vi "SA save Screenshot.vi"(8 "error in (no error)":errorcluster caption="에러 입력(에러 없음)", 10 "File Name":string, 11 "Instrument Manager 입력":refnum<class "Instrument Manager.lvclass">) -> (0 "error out":errorcluster caption="에러 출력", 3 "Instrument Manager 출력":refnum<class "Instrument Manager.lvclass">)   [LabVIEW 2023, in "Instrument Manager.lvclass"]
uses:
  Instrument Manager.lvclass
  Instrument Manager.lvclass/Instrument Manager.ctl
  Module/Spectrum Analyzer/Interface_Spectrum/Interface_Spectrum.lvclass
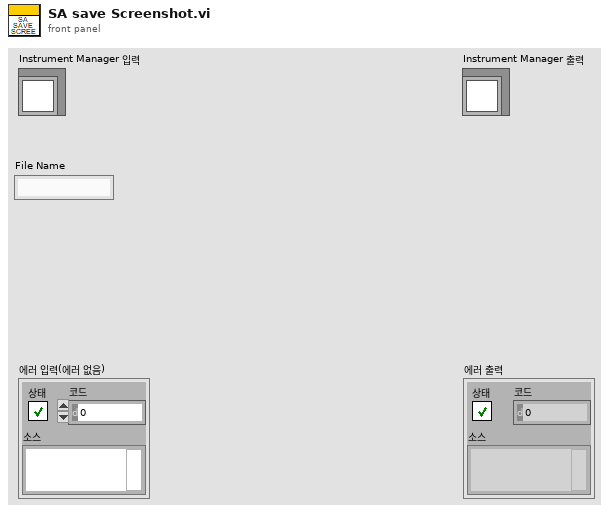
[diagram p1: front panel]
types:
  T1 = cluster{"Anritsu Call Box":refnum<class "Anritsu Call Box.lvclass">, "Spectrum Analyzer":refnum<class "Interface_Spectrum.lvclass">, "RF Switch Box":refnum<class "RF Filter Box.lvclass">, "Turn Table":refnum<class "Interface - Turn Table.lvclass">, "Mast":refnum<class "Interface - Mast.lvclass">, "3D Controller":refnum<class "Interface_3D Controller.lvclass">}
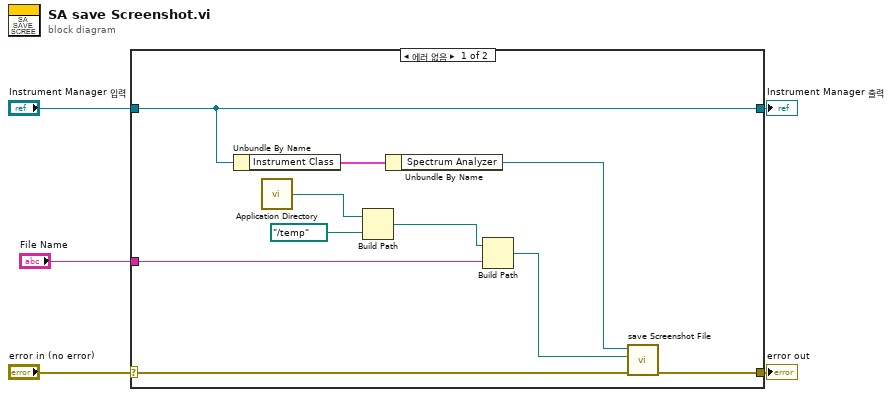
[diagram p0: block diagram]
diagram:
  n1 = case shown="에러 없음" "error in (no error)" {
    selector: "error in (no error)" -> [w12 w17]
    tunnel: [w11 w17] -> w4
    tunnel: [w10 w16] -> w2
    tunnel: "Instrument Manager 입력" -> [w10 w16]
    tunnel: "File Name" -> [w13 _]
    frame No Error {
      n2 = Unbundle By Name(w10) -> ("Instrument Class"=w15:T1)
      n3 = call <vilib>:"Application Directory.vi"() -> ("Application Directory"=w7:path)
      n4 = Build Path(base path=w7, name or relative path=path "../temp" ("이름 또는 상대 경로")) -> (appended path=w6:path)
      n5 = Unbundle By Name(w15) -> ("Spectrum Analyzer"=w14:refnum<class "Interface_Spectrum.lvclass">)
      n6 = Build Path(base path=w6, name or relative path=w13) -> (appended path=w8:path)
      n7 = call-dynamic "save Screenshot File.vi"("error in (no error)"=w12, "File Path"=w8, "Interface_Spectrum in"=w14) -> ("error out"=w11:errorcluster)  [unwired: 7 in, 1 out]
    }
    frame Error {
    }
  }
  "error out" <- w4
  "Instrument Manager 출력" <- w2
